vi "ClearOverlay.vi"(7 "Groups":string[](array[string]), 8 "error in":errorcluster, 11 "Image Reference In":T1) -> (0 "error out":errorcluster, 3 "Image Reference Out":T1)   [LabVIEW 2020, in "OpenLvVision_Overlays.lvlib"]
doc: "Clear all overlays or specific if a group is defined."
uses:
  OpenLvVision_Overlays.lvlib
  <vilib>/OpenLvVision/OpenLvVision_Image/Management/TypeDef/OLV Image.ctl
  <vilib>/OpenLvVision/OpenLvVision_Image/Management/OLV Management.lvlib
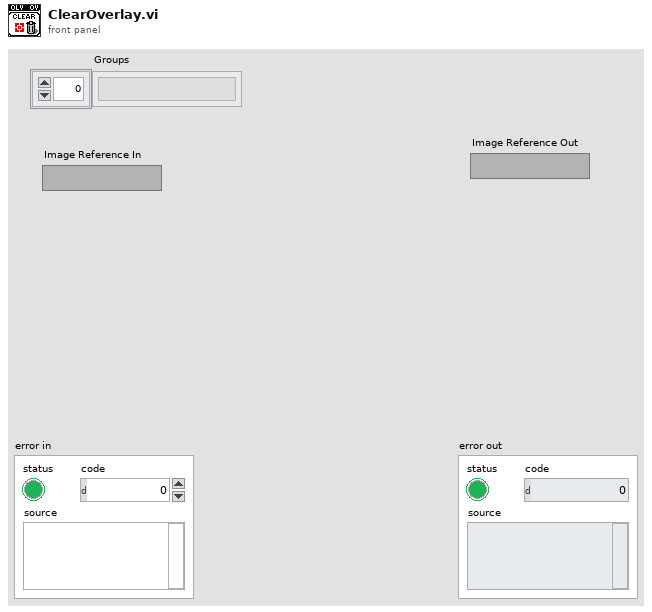
[diagram p1: front panel]
types:
  T1 = typedef "OLV OpenLvVision_Image.lvlib/OLV Management.lvlib/OLV Image.ctl" = refnum<image>
  T2 = typedef "IMAQ Image.ctl" = refnum<image>
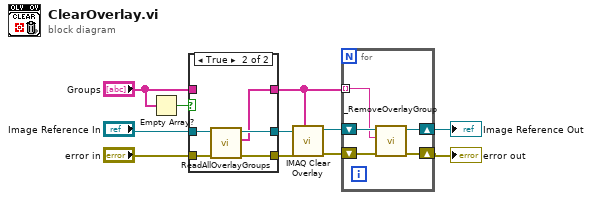
[diagram p0: block diagram]
diagram:
  n1 = Empty Array?(array="Groups") -> (empty?=w4:bool)
  n2 = case shown="True" w4 {
    tunnel: "error in" -> [w13 w19]
    tunnel: "Image Reference In" -> [w14 w18]
    tunnel: [w14 w17] -> w5
    tunnel: "Groups" -> [w12 _]
    tunnel: [w13 w16] -> w2
    tunnel: [w12 w15] -> w1
    frame False {
    }
    frame True {
      n3 = call "ReadAllOverlayGroups.vi"("error in"=w19, "Image Reference In"=w18) -> ("error out"=w16:errorcluster, "OverlayGroups"=w15:string[], "Image Reference Out"=w17:T1)  [unwired: 7 in]
    }
  }
  n4 = call "IMAQ Clear Overlay"("Groups"=w1, "error in (no error)"=w2, "Image"=w5) -> ("error out"=w11:errorcluster, "Image Out"=w10:T2)  [unwired: 7 in]
  n5 = for {
    shift-right: [w21] -> w9
    shift-left: w11 -> [w22]
    shift-right: [w23] -> w8
    shift-left: w10 -> [w24]
    tunnel: w1 -> [w20] mode=indexing
    n6 = call "_RemoveOverlayGroup.vi"("error in"=w22, "GroupName"=w20, "Image Reference In"=w24) -> ("error out"=w21:errorcluster, "Image Reference Out"=w23:T1)  [unwired: 7 in]
  }
  "error out" <- w9
  "Image Reference Out" <- w8
